vi "Get SLSC Chassis ID.vi"(8 "error in (no error)":errorcluster, 11 "SLSC Chassis Ref in":T2 format="%.0x") -> (0 "error out":errorcluster, 2 "SLSC Chassis ID":T1 {"chassisType" items=["e12001_CHASSIS_TYPE"]; "ChassisIDType" items=["ChassisName", "HostnameIPAddress"]}, 3 "SLSC Chassis Ref out":T2 format="%.0x")   [LabVIEW 2020, in "VeriStand SLSC Scripting.lvlib"]
uses:
  VeriStand SLSC Scripting.lvlib
  <vilib>/NI VeriStand/Custom Device API/Custom Device Item Ref.ctl
  Controls/SLSC Chassis ID.ctl
  NationalInstruments.VeriStand.SystemDefinitionAPI
  <vilib>/NI VeriStand/Custom Device API/Custom Device API.lvlib
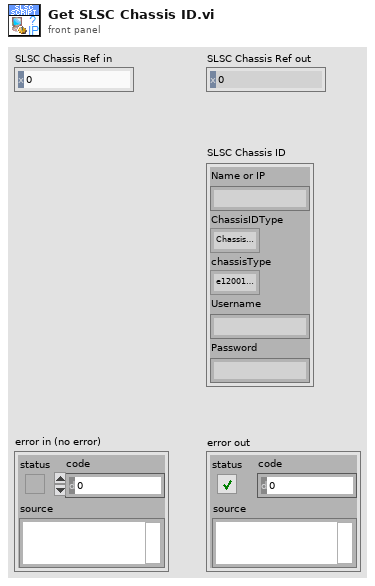
[diagram p1: front panel]
types:
  T1 = typedef "VeriStand SLSC Scripting.lvlib/SLSC Chassis ID.ctl" = cluster{"Name or IP":string, "ChassisIDType":i32, "chassisType":i32, "Username":string, "Password":string}
  T2 = typedef "Custom Device API.lvlib/Custom Device Item Ref.ctl" = u64
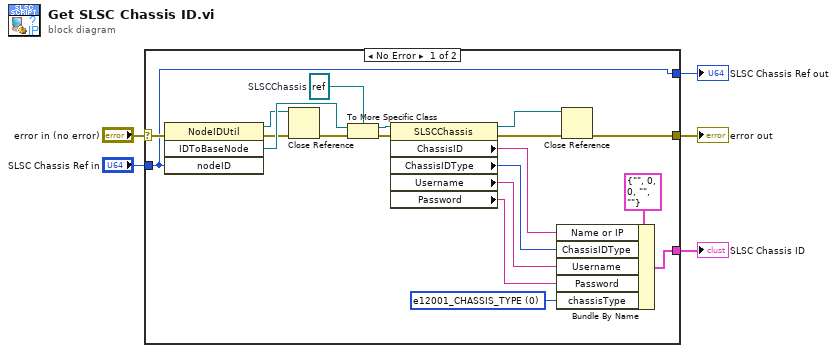
[diagram p0: block diagram]
diagram:
  n1 = case shown="No Error" "error in (no error)" {
    selector: "error in (no error)" -> [w15 w26]
    tunnel: [w19 w26] -> w5
    tunnel: "SLSC Chassis Ref in" -> [w14 w25]
    tunnel: [w14 w25] -> w2
    tunnel: [w12 _] -> w1
    frame No Error {
      w8 = 0 items=["e12001_CHASSIS_TYPE"] ("chassisType")
      w24 = refnum<k24> refnum  # SLSCChassis
      n2 = invoke class="NodeIDUtil" method="IDToBaseNode"(error in=w15, "nodeID"=w14) -> (reference out=w20:refnum<k24>, error out=w21:errorcluster, "IDToBaseNode"=w23:refnum<k24>)  [unwired: 2 in, 1 out]
      n3 = Close Reference(reference=w20, error in (no error)=w21) -> (error out=w22:errorcluster)
      n4 = To More Specific Class(target class=w24, reference=w23, error in=w22) -> (specific class reference=w10:refnum<k24>, error out=w18:errorcluster)
      n5 = property class="SLSCChassis"(reference=w10, error in=w18) -> (reference out=w17:refnum<k24>, error out=w16:errorcluster, "ChassisID"=w11:string, "ChassisIDType"=w9:i32, "Username"=w7:string, "Password"=w6:string)
      n6 = Bundle By Name(cluster=T1 {"Name or IP"="", "ChassisIDType"=0, "chassisType"=0, "Username"="", "Password"=""} ("SLSC Chassis ID"), "Name or IP"=w11, "ChassisIDType"=w9, "Username"=w7, "Password"=w6, "chassisType"=w8) -> (w12:T1)
      n7 = Close Reference(reference=w17, error in (no error)=w16) -> (error out=w19:errorcluster)
    }
    frame Error {
    }
  }
  "error out" <- w5
  "SLSC Chassis Ref out" <- w2
  "SLSC Chassis ID" <- w1
